vi "BB Raw Writer from Refnum.vi"(3 "BB Raw Writer Refnum":T1 {"refnum" format="%.0x"}) -> (5 "BB Raw Writer U64":u64)   [LabVIEW 2021, in "Iceoryx.lvlib"]
uses:
  Iceoryx.lvlib
  Typedef/BB Raw Writer Refnum.ctl
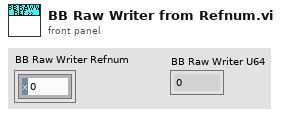
[diagram p1: front panel]
types:
  T1 = typedef "Iceoryx.lvlib/BB Raw Writer Refnum.ctl" = cluster{"refnum":u64, "BB Raw Writer":enum8{"bb_raw_writer"}}
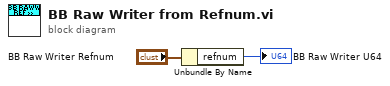
[diagram p0: block diagram]
diagram:
  n1 = Unbundle By Name("BB Raw Writer Refnum") -> ("refnum"=→"BB Raw Writer U64":u64)
